vi "Cached Tool List.vi"(8 "error in":errorcluster, 10 "server id in":i32, 11 "message json":string) -> (0 "error out":errorcluster, 3 "response":string)   [LabVIEW 2020, in "MCP Server.lvlib"]
doc: "Answers tools/list like tool list.vi, but builds the list of tools only when the tools of the server have changed. Same connector pane as tool list.vi: Handle Server Request.vi (tools/list) and Finish Tool Call Response.vi (which looks up the tool names for its \"Unknown tool\" message) call this VI instead.\n\nWhy: tool list.vi reads every tool VI through VI Server (connector pane, front panel controls, their labels, descriptions and limits) and builds the JSON schema of every input and output on each call. Requests are handled one at a time, so that time delays every other request too.\n\nHow: the key of the cache is the flattened Tools array of the server (Get Tools.vi), which holds everything Add Tool.vi stored: names, descriptions, inputs, outputs, titles, annotations and the VI references. When Tool List Cache.vi has a result for this server and this key, the response is made from it with the id of the request (Build Response Message.vi). Otherwise tool list.vi builds the response, and its result is stored, but only when it is not an error and the Tools array is still the same after the build. Add Tool.vi and Clear Tools.vi change the Tools array and therefore the key, so the next tools/list is built again: nothing has to invalidate the cache.\n\nNot noticed: a change made inside a tool VI (for example a control description) after Add Tool.vi. tool list.vi read those on every call; now they are read when the tool list is built, that is after the tools of the server changed."
uses:
  MCP Server.lvlib
  <vilib>/JDP Science/JSONtext/Next JSON Value.vi
  <vilib>/JDP Science/JSONtext/String Subset.vi
  <vilib>/JDP Science/JSONtext/Parsing/Advance past next JSON Value (inlined COPY).vi
  <vilib>/JDP Science/JSONtext/Parsing/Advance past whitespace.vi
  <vilib>/JDP Science/JSONtext/Parsing/Advance past String.vi
  <vilib>/JDP Science/JSONtext/Parsing/Advance past Number.vi
  <vilib>/JDP Science/JSONtext/Parsing/Advance past Line Ending.vi
  <vilib>/JDP Science/JSONtext/Parsing/Parse Full Path or Item Name.vi
  <vilib>/JDP Science/JSONtext/Parsing/Advance past Array.vi
  <vilib>/JDP Science/JSONtext/Parsing/Advance past Object.vi
  <vilib>/JDP Science/JSONtext/support/Error Cluster From Code.vi
  <vilib>/JDP Science/JSONtext/Offset/Find Item Locations by Path.vi
  <vilib>/JDP Science/JSONtext/JSONtext.lvlib
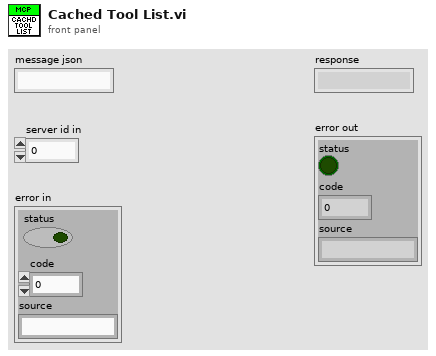
[diagram p1: front panel]
types:
  T1 = typedef "MCP Server.lvlib/Tool Data.ctl" = cluster{"Name":string, "Description":string, "Ignored":string[], "inputs":T2[], "outputs":T3[], "VI Refnum":refnum<vi>, "title":string, "annotations":T4}
  T2 = typedef "MCP Server.lvlib/Input Parameter.ctl" = cluster{"name":string, "type":string, "description":string, "required":bool, "raw name":string, "sub type":string, "array dimension":i32}
  T3 = typedef "MCP Server.lvlib/Output Parameter.ctl" = cluster{"name":string, "description":string, "type":string, "raw name":string}
  T4 = typedef "MCP Server.lvlib/Tool Annotations.ctl" = cluster{"readOnlyHint":T5, "destructiveHint":T5, "idempotentHint":T5, "openWorldHint":T5}
  T5 = typedef "MCP Server.lvlib/Tool Hint.ctl" = enum16{"not set", "true", "false"}
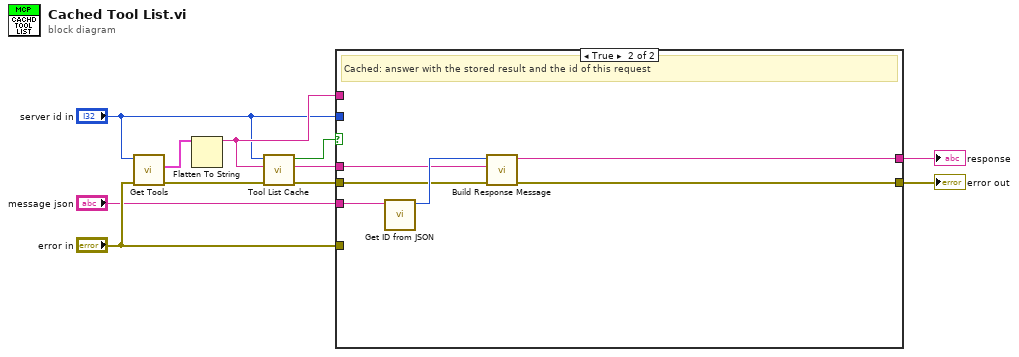
[diagram p0: block diagram]
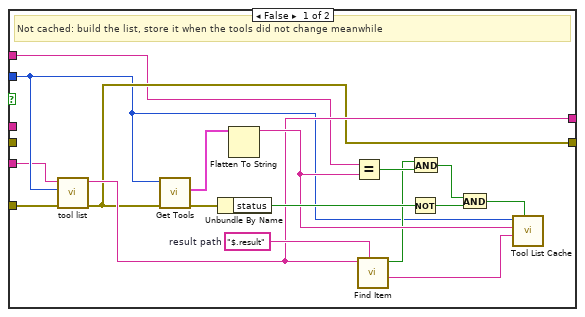
[diagram p2: hidden frame]
diagram:
  n1 = call "Get Tools.vi"("error in (no error)"="error in", "server id in"="server id in") -> ("error out"=w4:errorcluster, "Tools"=w5:T1[])  [unwired: 7 in, 1 out]
  n2 = Flatten To String(anything=w5) -> (data string=w6:string)  [unwired: 3 in, 2 out]
  n3 = call "Tool List Cache.vi"("error in"=w4, "key"=w6, "server id"="server id in") -> ("error out"=w9:errorcluster, "tools json out"=w8:string, "found?"=w7:bool)  [unwired: 6 in]
  n4 = case shown="True" w7 {
    tunnel: "message json" -> [w12 w29]
    tunnel: "server id in" -> [w13 _]
    tunnel: "error in" -> [w14 _]
    tunnel: w6 -> [w15 _]
    tunnel: w8 -> [_ w30]
    tunnel: w9 -> [_ w31]
    tunnel: [w17 w34] -> w10
    tunnel: [w16 w33] -> w11
    frame False {
      w18 = "$.result"  # result path
      # "Not cached: build the list, store it when the tools did not change meanwhile"
      n5 = call "tool list.vi"("error in"=w14, "server id in"=w13, "message json"=w12) -> ("error out"=w16:errorcluster, "response"=w17:string)  [unwired: 7 in]
      n6 = call "Get Tools.vi"("error in (no error)"=w16, "server id in"=w13) -> ("error out"=w21:errorcluster, "Tools"=w22:T1[])  [unwired: 7 in, 1 out]
      n7 = Unbundle By Name(w21) -> ("status"=w25:bool)
      n8 = Flatten To String(anything=w22) -> (data string=w23:string)  [unwired: 3 in, 2 out]
      n9 = Equal?(x=w15, y=w23) -> (x = y?=w24:bool)
      n10 = call <vilib>:"Find Item.vi"("$Path or Item Name"=w18, "JSON"=w17) -> ("<JSON>"=w19:string, "Found"=w20:bool)  [unwired: 6 in, 2 out]
      n11 = Not(x=w25) -> (.not. x?=w26:bool)
      n12 = And(x=w20, y=w24) -> (x .and. y?=w27:bool)
      n13 = And(x=w27, y=w26) -> (x .and. y?=w28:bool)
      n14 = call "Tool List Cache.vi"("write? (F)"=w28, "tools json"=w19, "key"=w23, "server id"=w13) -> ()  [unwired: 5 in, 3 out]
    }
    frame True {
      # "Cached: answer with the stored result and the id of this request"
      n15 = call "Get ID from JSON.vi"("message json"=w29) -> ("Data out"=w32:i32)  [unwired: 10 in]
      n16 = call "Build Response Message.vi"("error in (no error)"=w31, "Result content"=w30, "message id in"=w32) -> ("error out"=w33:errorcluster, "MCP message out"=w34:string)  [unwired: 7 in]
    }
  }
  "response" <- w10
  "error out" <- w11
